vi "CSM - Module Status.vi"(8 "Error In":errorcluster caption="error in (no error)", 11 "CSM Name":string) -> (0 "error out":errorcluster, 1 "#Nodes":i32, 2 "Mode":T1=enum."Stand Alone", 3 "CSM Name (Dup)":string, 4 "#Elements In Queue":i32)   [LabVIEW 2017, in "Communicable State Machine.lvlib"]
doc: "Obtains the status of a CSM module, including operation mode, number of workers, and number of messages pending in the message queue.\n\n\n> [!NOTE] <b>CSM Operation Modes</b>\n>\n> - <b>Stand-alone</b>: Independent operation mode. If no module name is specified, a random ID is automatically generated to identify the module.\n> - <b>CSM</b>: Normal CSM module.\n> - <b>Action Worker</b>: Worker Mode. Append `#` to the module name to mark this module as a worker. This module shares the same message queue with other workers having the same name.\n> - <b>Chain Node</b>: Chain node. Append `$` to the module name to mark this module as a chain node. Messages on the same chain will be passed sequentially until a node processes the message.\n\n\n-- <b>Controls</b> --\n- <b>CSM Name</b>: CSM module name.\n\n-- <b>Indicators</b> --\n- <b>CSM Name (dup)</b>: A copy of the input CSM module name.\n- <b>Mode</b>: Returns the operation mode of the module.\n- <b>#Nodes</b>: Number of nodes in Worker Mode or Chain of Responsibility Mode.\n- <b>#Elements In Queue</b>: Number of messages pending processing in the CSM message queue."
uses:
  Communicable State Machine.lvlib
  _Support/Typedef/_CSM_MODE.ctl
  _Support/CSMQ/_CSMOFGVOPER.ctl
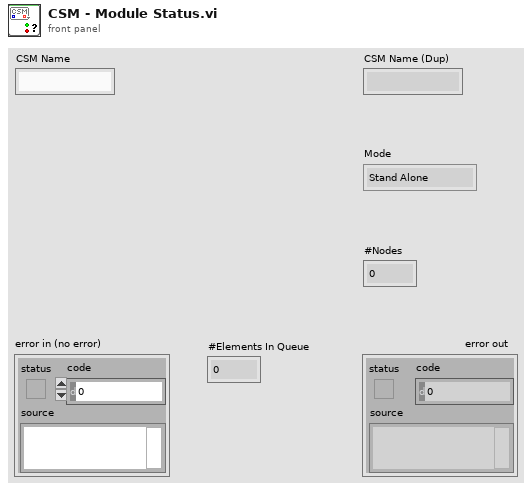
[diagram p1: front panel]
types:
  T1 = typedef "Communicable State Machine.lvlib/_CSM_MODE.ctl" = enum16{"Not Exist", "Stand Alone", "CSM", "Worker", "Worker Agent", "Chain Node", "Chain"}
  T2 = typedef "Communicable State Machine.lvlib/_CSMOFGVOPER.ctl" = enum16{"Create If not Exist", "Get By Name", "List", "Check If Name Exists", "Release", "Module Status", "Create Status Event Handler", "Destroy Status Event Handler", "Clear Invalid Objs"}
  T3 = typedef "Communicable State Machine.lvlib/_CSMObj.ctl" = cluster{"info":T4, "Refs":T5}
  T4 = typedef "Communicable State Machine.lvlib/_CSMObj-Info.ctl" = cluster{"Module Name":string, "Requested Name":string, "Group Name":string, "Mode":T1, "Allowed Messages":string[]}
  T5 = typedef "Communicable State Machine.lvlib/_CSMObj-Refs.ctl" = cluster{"WatchDogQ":refnum<queue>, "CSMDataDVR":refnum<data-value>, "Queue":T6, "GroupDataDVR":refnum<data-value>, "TagMap":refnum<data-value>, "ExitEvent":refnum<user-event>, "NewStateEvent":refnum<user-event>, "StatusEvent":refnum<user-event>, "InterruptEvent":refnum<user-event>}
  T6 = typedef "Communicable State Machine.lvlib/Priority Queue.ctl" = cluster{"HPriorityQ":refnum<queue>, "LowPriorityQ":refnum<queue>}
  T7 = typedef "Communicable State Machine.lvlib/_CSMObj-ModeData.ctl" = cluster{"CSMDataDVR":refnum<data-value>[], "PriorityQueues":T6[], "Messages of Chain Nodes":cluster{"Module Name":string, "Allowed Messages":string[]}[], "Chain Message Mapping Map":variant, "SharedRegistryRules":string[]}
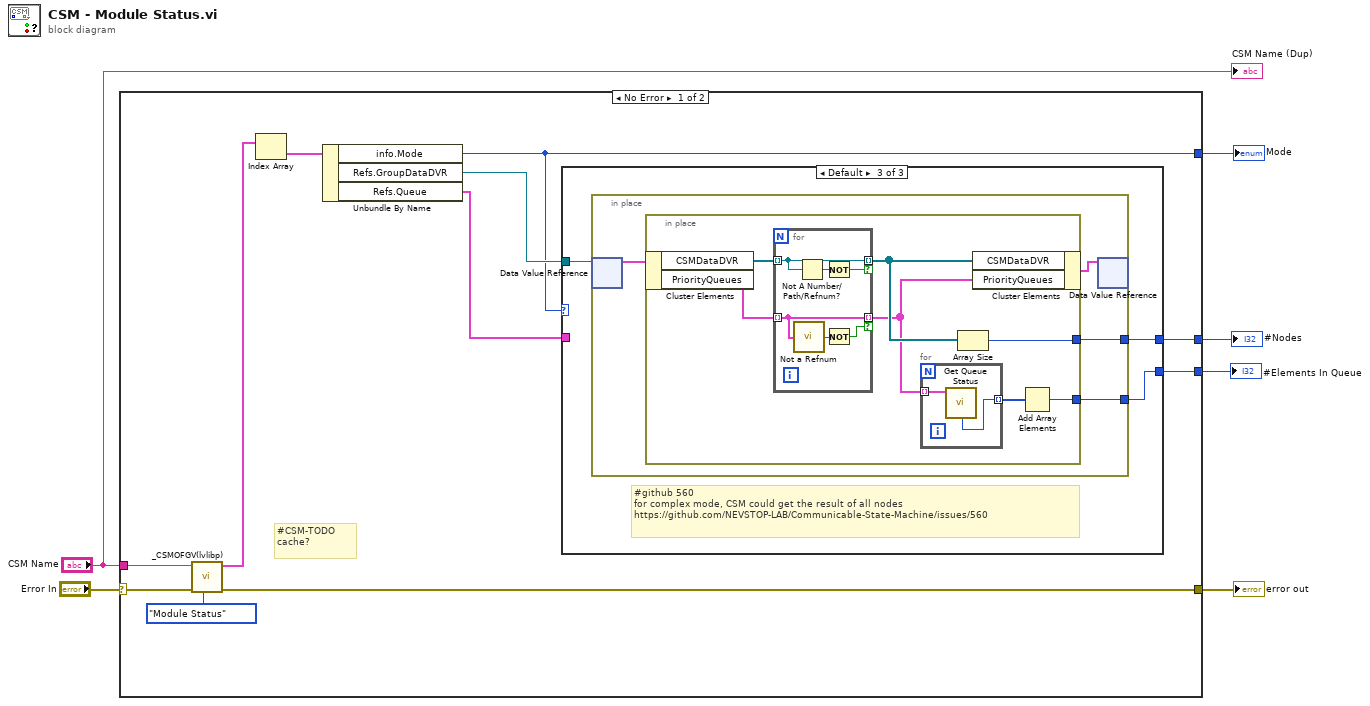
[diagram p0: block diagram]
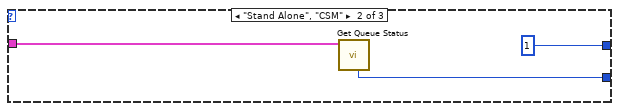
[diagram p3: hidden frame]
diagram:
  n1 = case shown="No Error" "Error In" {
    selector: "Error In" -> [w17 w43]
    tunnel: [w16 w43] -> w5
    tunnel: [w9 _] -> w4
    tunnel: "CSM Name" -> [w12 _]
    tunnel: [w10 _] -> w2
    tunnel: [w7 _] -> w1
    frame No Error {
      # "#CSM-TODO\ncache?"
      n2 = call "_CSMOFGV(lvlibp).vi"("Operation"=_CSMOFGVOPER."Module Status", "Error In"=w17, "Name (\"\" to Use UUID) In"=w12) -> ("error out"=w16:errorcluster, "Array"=w14:T3[])  [unwired: 6 in, 1 out]
      n3 = Index Array(array=w14) -> (element=w13:T3)  [unwired: 1 in]
      n4 = Unbundle By Name(w13) -> ("info.Mode"=w9:T1, "Refs.GroupDataDVR"=w11:refnum<data-value>, "Refs.Queue"=w8:T6)
      n5 = case shown="Default" w9 {
        tunnel: w11 -> [_ _ w23]
        tunnel: [_ 1 w22] -> w10
        tunnel: w8 -> [_ w20 _]
        tunnel: [_ w19 w21] -> w7
        frame "Not Exist" {
        }
        frame "Stand Alone", "CSM" {
          n6 = call "Get Queue Status.vi"("Priority Queue In"=w20) -> ("# Elements In Queue"=w19:i32)  [unwired: 6 in, 4 out]
        }
        frame Default {
          # "#github 560\nfor complex mode, CSM could get the result of all nodes \nhttps://github.com/NEVSTOP-LAB/Communicable-State-Machine/issues/560"
          n7 = in-place {
            in-place-border: [w25] -> w22
            in-place-border: [w24] -> w21
            n8 = in-place-dvr #1(w23) -> (w27:T7)  [unwired: 1 out]
            n9 = in-place {
              in-place-border: [w33] -> w25
              in-place-border: [w28] -> w24
              n10 = in-place-cluster #2(w27) -> ("CSMDataDVR"=w34:refnum<data-value>[], "PriorityQueues"=w31:T6[])
              n11 = for {
                tunnel: [w42] -> w32 mode=indexing if=w40
                tunnel: w34 -> [w42] mode=indexing
                tunnel: w31 -> [w39] mode=indexing
                tunnel: [w39] -> w30 mode=indexing if=w37
                n12 = call "Not a Refnum.vi"("Priority Queue.lvclass"=w39) -> ("NaN/Path/Refnum?"=w38:bool)  [unwired: 4 in]
                n13 = Not A Number/Path/Refnum?(number/path/refnum=w42) -> (NaN/Path/Refnum?=w41:bool)
                n14 = Not(x=w41) -> (.not. x?=w40:bool)
                n15 = Not(x=w38) -> (.not. x?=w37:bool)
              }
              n16 = for {
                tunnel: w30 -> [w36] mode=indexing
                tunnel: [w35] -> w29 mode=indexing
                n17 = call "Get Queue Status.vi"("Priority Queue In"=w36) -> ("# Elements In Queue"=w35:i32)  [unwired: 6 in, 4 out]
              }
              n18 = Array Size(array=w32) -> (size(s)=w33:i32)
              n19 = in-place-cluster #2("CSMDataDVR"=w32, "PriorityQueues"=w30) -> (w26:T7)
              n20 = Add Array Elements(numeric array=w29) -> (sum=w28:i32)
            }
            n21 = in-place-dvr #1(w26) -> ()  [unwired: 2 out]
          }
        }
      }
    }
    frame Error {
    }
  }
  "error out" <- w5
  "Mode" <- w4
  "#Nodes" <- w2
  "#Elements In Queue" <- w1
  "CSM Name (Dup)" <- "CSM Name"
